vi "Get Driver List - Multiple Converter.vi"(11 "error in":errorcluster) -> (15 "error out":errorcluster)   [LabVIEW 2021, in "Converter.lvlib"]
uses:
  Converter.lvlib
  <vilib>/Utility/traverseref.llb/TRef TravTarget.ctl
  <vilib>/Utility/traverseref.llb/VI Scripting - Traverse.lvlib
  Converter Reusables/Converter Reusables.lvlib
  Path Functions/Path Functions.lvlib
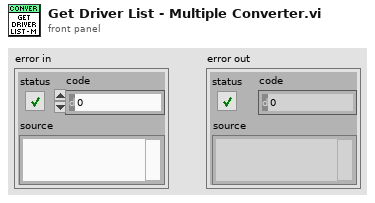
[diagram p1: front panel]
types:
  T1 = typedef "TRef TravTarget.ctl" = enum16{"FP", "BD", "Other"}
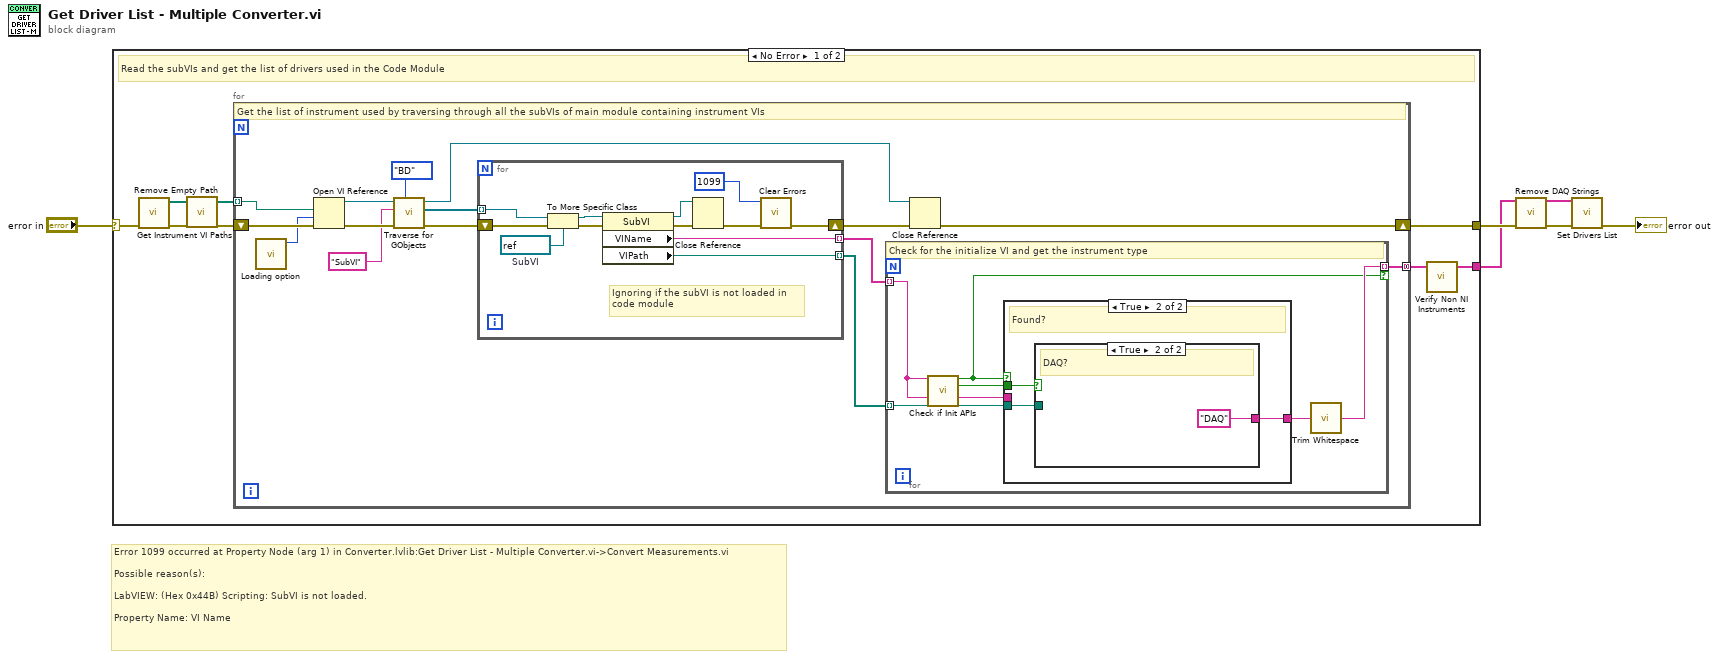
[diagram p0: block diagram]
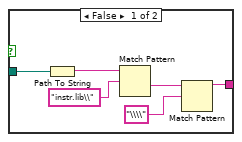
[diagram p3: hidden frame]
diagram:
  # "Error 1099 occurred at Property Node (arg 1) in Converter.lvlib:Get Driver List - Multiple Converter.vi->Convert Measurements.vi\n\nPossible reason(s):\n\nLabVIEW: (Hex 0x44B) Scripting: SubVI is not loaded.\n\nProperty Name: VI Name"
  n1 = case shown="No Error" "error in" {
    selector: "error in" -> [w11 w56]
    tunnel: [w7 w56] -> w4
    tunnel: [w8 _] -> w2
    frame No Error {
      # "Read the subVIs and get the list of drivers used in the Code Module"
      n2 = call "Get Instrument VI Paths.vi"("error in"=w11) -> ("error out"=w10:errorcluster, "instr vi paths[]"=w12:path[])  [unwired: 9 in]
      n3 = call "Remove Empty Path.vi"("instr vi paths in"=w12) -> ("instr vi paths out"=w6:path[])  [unwired: 4 in]
      n4 = for {
        tunnel: w6 -> [w22] mode=indexing
        tunnel: [w18] -> w9 mode=concatenating
        shift-right: [w16] -> w7
        shift-left: w10 -> [w21]
        # "Get the list of instrument used by traversing through all the subVIs of main module containing instrument VIs"
        n5 = call "Loading option.vi"() -> ("options"=w13:i32)  [unwired: 11 in]
        n6 = Open VI Reference(vi path=w22, options=w13, error in (no error)=w21) -> (vi reference=w17:refnum<vi>, error out=w25:errorcluster)  [unwired: 3 in]
        n7 = call <vilib>:"Traverse for GObjects.vi"("Traverse Target"=TRef_TravTarget."BD", "error in (no error)"=w25, "Class Name"="SubVI", "VI Refnum"=w17) -> ("error out"=w27:errorcluster, "References"=w26:refnum<vi>[], "dup VI Refnum"=w14:refnum<vi>)  [unwired: 4 in, 1 out]
        n8 = for {
          tunnel: w26 -> [w54] mode=indexing
          tunnel: [w50] -> w20 mode=indexing
          tunnel: [w49] -> w19 mode=indexing
          shift-right: [w45] -> w15
          shift-left: w27 -> [w53]
          w55 = refnum<vi> refnum  # SubVI
          # "Ignoring if the subVI is not loaded in\ncode module"
          n9 = To More Specific Class(target class=w55, reference=w54, error in=w53) -> (specific class reference=w52:refnum<vi>, error out=w51:errorcluster)
          n10 = property class="SubVI"(reference=w52, error in=w51) -> (reference out=w48:refnum<vi>, error out=w47:errorcluster, "VIName"=w50:string, "VIPath"=w49:path)
          n11 = Close Reference(reference=w48, error in (no error)=w47) -> (error out=w46:errorcluster)
          n12 = call <vilib>:"Clear Errors.vi"("error in (no error)"=w46, "specific error code to clear (0: all)"=1099) -> ("error out"=w45:errorcluster)  [unwired: 4 in, 1 out]
        }
        n13 = for {
          tunnel: w20 -> [w29] mode=indexing
          tunnel: w19 -> [w33] mode=indexing
          tunnel: [w32] -> w18 mode=indexing if=w30
          # "Check for the initialize VI and get the instrument type"
          n14 = call "Check if Init APIs.vi"("vi name"=w29) -> ("instrument driver found?"=w30:bool, "daq?"=w28:bool)  [unwired: 13 in]
          n15 = case shown="True" w30 {
            tunnel: w33 -> [_ w36]
            tunnel: [_ w35] -> w31
            tunnel: w29 -> [_ _]
            tunnel: w28 -> [_ w34]
            frame False {
            }
            frame True {
              # "Found?"
              n16 = case shown="True" w34 {
                tunnel: w36 -> [w38 _]
                tunnel: [w37 "DAQ"] -> w35
                frame False {
                  n17 = Path To String(path=w38) -> (string=w39:string)
                  n18 = Match Pattern(string=w39, regular expression="instr.lib\\") -> (after substring=w41:string)  [unwired: 1 in, 3 out]
                  n19 = Match Pattern(string=w41, regular expression="\\\\") -> (before substring=w37:string)  [unwired: 1 in, 3 out]
                }
                frame True {
                  # "DAQ?"
                }
              }
            }
          }
          n20 = call <vilib>:"Trim Whitespace.vi"("string"=w31) -> ("trimmed string"=w32:string)  [unwired: 1 in]
        }
        n21 = Close Reference(reference=w14, error in (no error)=w15) -> (error out=w16:errorcluster)
      }
      n22 = call "Verify Non NI Instruments.vi"("instrument types in"=w9) -> ("instrument types out"=w8:string[])  [unwired: 4 in]
    }
    frame Error {
    }
  }
  n23 = call "Remove DAQ Strings.vi"("instrument types in"=w2) -> ("instrument types out"=w1:string[])  [unwired: 14 in]
  n24 = call "Set Drivers List.vi"("name"=w1, "error in"=w4) -> ("error out"=→"error out":errorcluster)  [unwired: 13 in]
